vi "G-Uart-Close.vi"(8 "error in (no error)":errorcluster caption="错误输入（无错误）", 11 "G-Uart-Class 输入":refnum<class "G-Uart-Class.lvclass">) -> (0 "error out":errorcluster caption="错误输出", 3 "G-Uart-Class 输出":refnum<class "G-Uart-Class.lvclass">)   [LabVIEW 2025, in "G-Uart-Class.lvclass"]
uses:
  G-Uart-Class.lvclass
panel:
  # "欢迎下次使用小高的串口类"
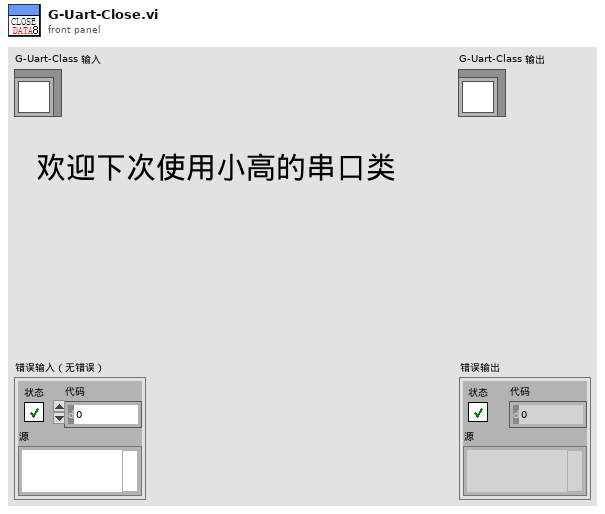
[diagram p1: front panel]
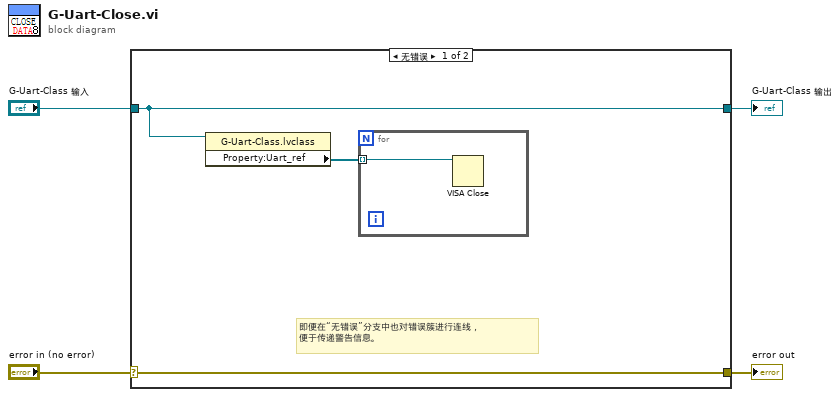
[diagram p0: block diagram]
diagram:
  n1 = case shown="无错误" "error in (no error)" {
    selector: "error in (no error)" -> [w7 w10]
    tunnel: [w7 w10] -> w3
    tunnel: [w6 w9] -> w1
    tunnel: "G-Uart-Class 输入" -> [w6 w9]
    frame No Error {
      # "即便在“无错误”分支中也对错误簇进行连线，\n便于传递警告信息。"
      n2 = property class="G-Uart-Class.lvclass"(reference=w6) -> ("Property:Uart_ref"=w5:refnum<visa-resource-name>[])  [unwired: 1 in, 2 out]
      n3 = for {
        tunnel: w5 -> [w8] mode=indexing
        n4 = VISA Close(VISA resource name=w8) -> ()  [unwired: 1 in, 1 out]
      }
    }
    frame Error {
    }
  }
  "error out" <- w3
  "G-Uart-Class 输出" <- w1
